vi "Signal Stopped.vi"(11 "Actor in":refnum<class "Sequence Executor.lvclass">) -> (3 "Actor out":refnum<class "Sequence Executor.lvclass">)   [LabVIEW 2026, in "Sequence Executor.lvclass"]
doc: "Stop Core hook (seriesAfter, after Call Parent). Sends TRUE on the Stopped Notification so the launcher's Wait on Notification returns."
uses:
  Sequence Executor.lvclass
  Sequence Executor.lvclass/Sequence Executor.ctl
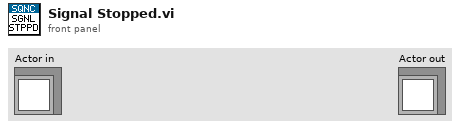
[diagram p1: front panel]
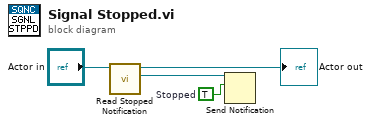
[diagram p0: block diagram]
diagram:
  w2 = TRUE  # Stopped
  n1 = call "Read Stopped Notification.vi"("Sequence Executor in"="Actor in") -> ("Stopped Notification"=w3:refnum<notifier>, "Sequence Executor out"=→"Actor out":refnum<class "Sequence Executor.lvclass">)  [unwired: 8 in, 1 out]
  n2 = Send Notification(notification=w2, notifier=w3) -> ()  [unwired: 1 in, 2 out]
